vi "VM Spy - Dialog - Context Name.vi"(11 "VC Handle":T1=-1) -> (0 "OK out":bool, 3 "dup VC Handle":T1=-1)   [LabVIEW 2021]
doc: "::: CalcExpress Toolkit :::\nCopyright (c) 2000-2026 Konstantin Shifershteyn. All rights reserved."
uses:
  vi.lib/addons/CalcExpress/cetypes.llb/VarMan Variable Context Handle.ctl
panel:
  in  "cancel":bool
  in  "set":bool
  in  "Context name":string
  out "Context handle":i32=-1
  # "*) an empty name makes the context be anonymous"
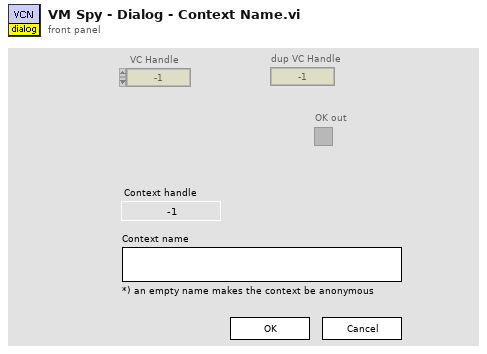
[diagram p1: front panel]
types:
  T1 = typedef "VarMan Variable Context Handle.ctl" = i32
  T2 = enum32{"nothing", "reset", "assign name", "get name", "get handle"}
  T3 = typedef "eventvkey.ctl" = enum16{"ASCII", "Enter", "Return", "Shift", "Ctrl", "Alt", "Cmd", "Opt", "Caps", "NumLock", "Clear", "Break", "Up", "Down", "Left", "Right", "Insert", "Delete", "Home", "End", "PageUp", "PageDown", "Escape", "Help", "Pause", "ScrollLock", "F1", "F2", "F3", "F4", "F5", "F6", "F7", "F8", "F9", "F10", "F11", "F12", "F13", "F14", "F15", "F16", "F17", "F18", "F19", "F20", "F21", "F22", "F23", "F24", "Play", "VolumeUp", "VolumeDown", "Mute", "Two Byte Char"}
  T4 = cluster{"Shift":bool, "Ctrl":bool, "Alt":bool, "Cmd":bool, "Opt":bool}
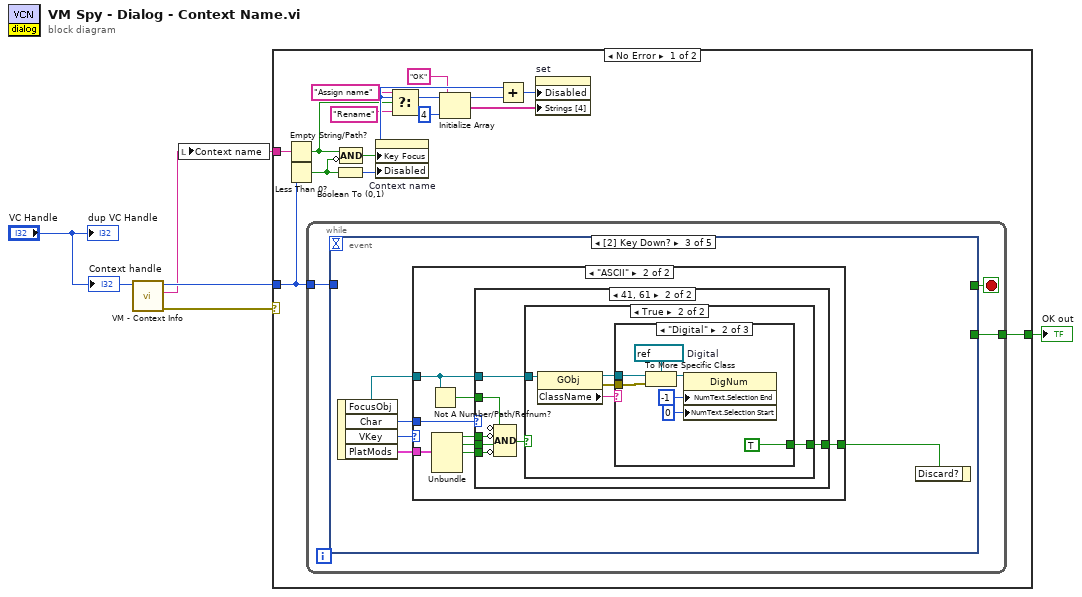
[diagram p0: block diagram]
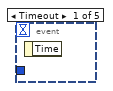
[diagram p2: hidden frame]
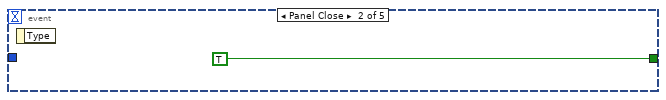
[diagram p3: hidden frame]
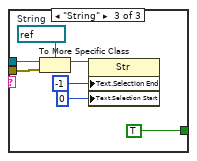
[diagram p8: hidden frame]
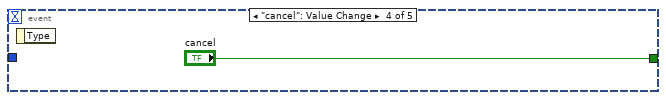
[diagram p9: hidden frame]
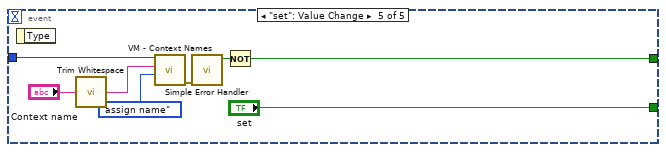
[diagram p10: hidden frame]
diagram:
  n1 = call "VM - Context Info.vi"("VC Handle"="VC Handle") -> ("error out"=w3:errorcluster, "VC Name"=w2:string, "dup VC Handle"=w4:T1)  [unwired: 6 in, 2 out]
  n2 = local write "Context name"(w2) -> ()
  n3 = case shown="No Error" w3 {
    tunnel: [w18 _] -> w5
    tunnel: w2 -> [w16 _]
    tunnel: w4 -> [w14 _]
    frame No Error {
      n4 = Empty String/Path?(string/path=w16) -> (empty?=w10:bool)
      n5 = Less Than 0?(x=w14) -> (x < 0?=w13:bool)
      n6 = while {
        tunnel: [w20] -> w18
        tunnel: w14 -> [w19]
        stop <- w21 stop-if-true
        n7 = event shown="[2] Key Down?" {
          selector: _ -> [_ _ _ _ _]
          dyn-events: _ -> [_ _ _ _ _]
          timeout: _ -> [_ _ _ _ _]
          tunnel: [_ TRUE _ "cancel" w66] -> w21
          tunnel: [_ _ _ _ "set"] -> w20
          tunnel: w19 -> [_ _ _ _ w64]
          event Timeout {
            n8 = event-data() -> ()  [unwired: 1 in, 1 out]
          }
          event Panel Close {
            n9 = event-data() -> ()  [unwired: 1 in, 1 out]
          }
          event Key Down? {
            n10 = event-data() -> ("FocusObj"=w23:refnum<vi>, "Char"=w24:i16, "VKey"=w25:T3, "PlatMods"=w26:T4)  [unwired: 1 in]
            n11 = case shown="\"ASCII\"" w25 {
              tunnel: w26 -> [_ w35]
              tunnel: [_ w29] -> w27
              tunnel: w24 -> [_ w31]
              tunnel: w23 -> [_ w30]
              frame Default {
              }
              frame "ASCII" {
                n12 = Not A Number/Path/Refnum?(number/path/refnum=w30) -> (NaN/Path/Refnum?=w28:bool)
                n13 = Unbundle(w35) -> ("Shift"=w34:bool, "Ctrl"=w33:bool, "Alt"=w32:bool)  [unwired: 2 out]
                n14 = case shown="41, 61" w31 {
                  tunnel: w34 -> [_ w42]
                  tunnel: w33 -> [_ w41]
                  tunnel: w32 -> [_ w40]
                  tunnel: w30 -> [_ w38]
                  tunnel: [_ w37] -> w29
                  tunnel: w28 -> [_ w36]
                  frame Default {
                  }
                  frame 65, 97 {
                    n15 = Compound Arithmetic op=AND(invert w36, invert w42, w41, invert w40) -> (w39:bool)
                    n16 = case shown="True" w39 {
                      tunnel: w38 -> [_ w47]
                      tunnel: [_ w45] -> w37
                      frame False {
                      }
                      frame True {
                        n17 = property class="GObj"(reference=w47) -> (reference out=w44:refnum<vi>, error out=w43:errorcluster, "ClassName"=w46:string)  [unwired: 1 in]
                        n18 = case shown="\"Digital\"" w46 {
                          tunnel: [_ TRUE TRUE] -> w45
                          tunnel: w44 -> [_ w52 w59]
                          tunnel: w43 -> [_ w51 w58]
                          frame Default {
                          }
                          frame "Digital" {
                            w53 = refnum<vi> refnum  # Digital
                            n19 = To More Specific Class(target class=w53, reference=w52, error in=w51) -> (specific class reference=w50:refnum<vi>)  [unwired: 1 out]
                            n20 = property class="DigNum"(reference=w50, "NumText.Selection End"=-1 ("Numeric Text.Selection:End"), "NumText.Selection Start"=u32 0 ("Numeric Text.Selection:Start")) -> ()  [unwired: 1 in, 2 out]
                          }
                          frame "String" {
                            w60 = refnum<vi> refnum  # String
                            n21 = To More Specific Class(target class=w60, reference=w59, error in=w58) -> (specific class reference=w57:refnum<vi>)  [unwired: 1 out]
                            n22 = property class="Str"(reference=w57, "Text.Selection End"=-1 ("Numeric Text.Selection:End"), "Text.Selection Start"=u32 0 ("Numeric Text.Selection:Start")) -> ()  [unwired: 1 in, 2 out]
                          }
                        }
                      }
                    }
                  }
                }
              }
            }
            n23 = event-data("Discard?"=w27) -> ()  [unwired: 1 in, 1 out]
          }
          event "cancel": Value Change {
            n24 = event-data() -> ()  [unwired: 1 in, 1 out]
          }
          event "set": Value Change {
            n25 = event-data() -> ()  [unwired: 1 in, 1 out]
            n26 = call <vilib>:"Trim Whitespace.vi"("string"="Context name") -> ("trimmed string"=w63:string)  [unwired: 1 in]
            n27 = call "VM - Context Names.vi"("action"=T2."assign name", "VC Name"=w63, "VC Handle"=w64) -> ("error out"=w69:errorcluster)  [unwired: 3 in, 3 out]
            n28 = call <vilib>:"Simple Error Handler.vi"("error in (no error)"=w69) -> ("error?"=w67:bool)  [unwired: 4 in, 4 out]
            n29 = Not(x=w67) -> (.not. x?=w66:bool)
          }
        }
      }
      n30 = Boolean To (0,1)(Boolean=w13) -> (0, 1=w12:i16)
      n31 = Compound Arithmetic op=AND(w10, invert w13) -> (w15:bool)
      n32 = property on="Context name" class="Str"("Key Focus"=w15, "Disabled"=w12) -> ()  [unwired: 2 in, 2 out]
      n33 = Select(t="Assign name", s=w10, f="Rename") -> ()  [unwired: 1 out]
      n34 = Initialize Array("OK", 4 ("dimension size")) -> (w7:string[])
      n35 = Add(x=w12, y=w12) -> (x+y=w17:i16)
      n36 = property on="set" class="Bool"("Disabled"=w17, "Strings [4]"=w7) -> ()  [unwired: 2 in, 2 out]
    }
    frame Error {
    }
  }
  "OK out" <- w5
  "Context handle" <- "VC Handle"
  "dup VC Handle" <- "VC Handle"
